vi "ReadRegister.vi"(6 "error in":errorcluster, 7 "string in":string, 9 "connection ID in":refnum<k5>) -> (0 "error out":errorcluster, 1 "number out":i32, 2 "string out":string, 3 "connection ID out":refnum<k5>, 4 "boolean array out":bool[](array[boolean]))   [LabVIEW 2014]
panel:
  out "row data out":string
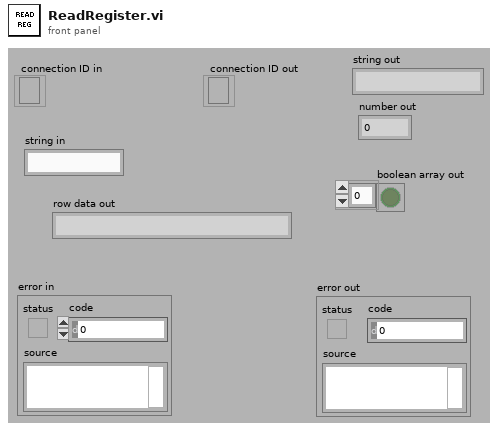
[diagram p1: front panel]
types:
  T1 = enum16{"Standard", "Buffered", "CRLF", "Immediate"}
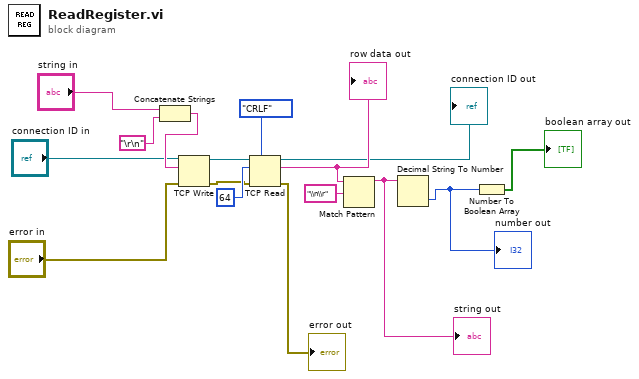
[diagram p0: block diagram]
diagram:
  n1 = Concatenate Strings("string in", "\r\n") -> (w14:string)
  n2 = TCP Write(connection ID="connection ID in", data in=w14, error in (no error)="error in") -> (connection ID out=w16:refnum<k5>, error out=w2:errorcluster)  [unwired: 1 in, 1 out]
  n3 = TCP Read(connection ID=w16, bytes to read=64, error in (no error)=w2, 7:T1."CRLF" ("mode (standard)")) -> (connection ID out=→"connection ID out":refnum<k5>, data out=w10:string, error out=→"error out":errorcluster)  [unwired: 1 in]
  "row data out" <- w10
  n4 = Match Pattern(string=w10, regular expression="\\n\\r") -> (before substring=w9:string)  [unwired: 1 in, 3 out]
  "string out" <- w9
  n5 = Decimal String To Number(string=w9) -> (number=w8:i32)  [unwired: 2 in, 1 out]
  "number out" <- w8
  n6 = Number To Boolean Array(number=w8) -> (Boolean array=→"boolean array out":bool[])
